vi "modify channel test.vi"() -> (0 "error out":errorcluster, 2 "channel modified?":bool)   [LabVIEW 2014, in "Shared Memory tests.lvlib"]
doc: "Tests the 'Replace Line' VI."
uses:
  Shared Memory tests.lvlib
  <vilib>/NI/Tag Bus Module Framework/channel/TBM channel.lvclass/TBM channel.ctl
  <vilib>/NI/Tag Bus Module Framework/channel/channel classification.ctl
  <vilib>/NI/Tag Bus/tag/tag descriptor.lvclass/tag descriptor.ctl
  <vilib>/NI/Tag Bus Module Framework/channel/Read channel classification.vi
  <vilib>/NI/Tag Bus Module Framework/channel/Write channel classification.vi
  module/configuration/Shared Memory configuration.lvclass
  <vilib>/NI/Tag Bus Module Framework/channel/TBM channel.lvclass
  <vilib>/NI/Tag Bus/tag/tag descriptor.lvclass
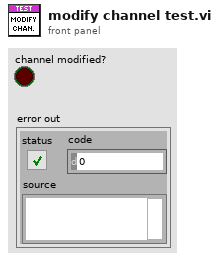
[diagram p1: front panel]
types:
  T1 = typedef "Shared Memory configuration.lvclass/Line.ctl" = cluster{"channel":refnum<class "TBM channel.lvclass">}
  T2 = typedef "TBM channel.lvclass/channel classification.ctl" = enum16{"input data", "output data", "processing parameter", "processing result"}
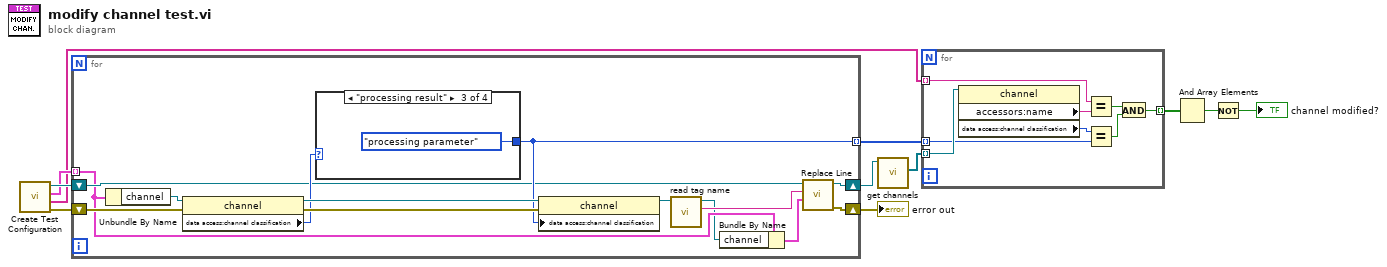
[diagram p0: block diagram]
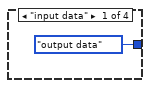
[diagram p2: hidden frame]
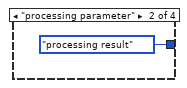
[diagram p3: hidden frame]
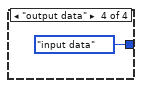
[diagram p4: hidden frame]
diagram:
  n1 = call "Create Test Configuration.vi"() -> ("error out"=w3:errorcluster, "channel names"=w2:string[], "Lines"=w4:T1[], "Module Configuration"=w5:refnum<class "Shared Memory configuration.lvclass">)  [unwired: 3 in, 5 out]
  n2 = for {
    shift-right: [w18] -> w11
    shift-left: w5 -> [w17]
    shift-right: [w19] -> w10
    shift-left: w3 -> [w25]
    tunnel: w4 -> [w16] mode=indexing
    tunnel: [w21] -> w6 mode=indexing
    n3 = Unbundle By Name(w16) -> ("channel"=w20:refnum<class "TBM channel.lvclass">)
    n4 = property class="channel"(reference=w20, error in=w25) -> (reference out=w23:refnum<class "TBM channel.lvclass">, error out=w24:errorcluster, "data access:channel classification"=w22:T2)
    n5 = case shown="\"processing result\"" w22 {
      tunnel: [channel_classification."output data" ("channel classification") channel_classification."processing result" ("channel classification") channel_classification."processing parameter" ("channel classification") channel_classification."input data" ("channel classification")] -> w21
      frame "input data" {
      }
      frame "processing parameter" {
      }
      frame "processing result" {
      }
      frame "output data" {
      }
    }
    n6 = property class="channel"(reference=w23, error in=w24, "data access:channel classification"=w21) -> (reference out=w13:refnum<class "TBM channel.lvclass">)  [unwired: 1 out]
    n7 = call <vilib>:"read tag name.vi"("system tag in"=w13) -> ("name"=w14:string, "system tag out"=w12:refnum<class "TBM channel.lvclass">)  [unwired: 8 in, 1 out]
    n8 = Bundle By Name(cluster=w16, "channel"=w12) -> (w15:T1)
    n9 = call "Replace Line.vi"("New Line"=w15, "Line Name"=w14, "Shared Memory configuration in"=w17) -> ("error out"=w19:errorcluster, "Shared Memory configuration out"=w18:refnum<class "Shared Memory configuration.lvclass">)  [unwired: 6 in, 1 out]
  }
  "error out" <- w10
  n10 = call-dynamic "get channels.vi"("Shared Memory configuration in"=w11) -> ("channels"=w9:refnum<class "TBM channel.lvclass">[])  [unwired: 9 in, 1 out]
  n11 = for {
    tunnel: w9 -> [w36] mode=indexing
    tunnel: [w35] -> w8 mode=indexing
    tunnel: w6 -> [w34] mode=indexing
    tunnel: w2 -> [w31] mode=indexing
    n12 = property class="channel"(reference=w36) -> ("accessors:name"=w32:string, "data access:channel classification"=w33:T2)  [unwired: 1 in, 2 out]
    n13 = Equal?(x=w31, y=w32) -> (x = y?=w30:bool)
    n14 = Equal?(x=w33, y=w34) -> (x = y?=w37:bool)
    n15 = And(x=w30, y=w37) -> (x .and. y?=w35:bool)
  }
  n16 = And Array Elements(Boolean array=w8) -> (logical AND=w7:bool)
  n17 = Not(x=w7) -> (.not. x?=→"channel modified?":bool)
